vi "Get All Methods.vi"(8 "error in (no error)":errorcluster) -> (0 "error out":errorcluster, 3 "Methods[]":T1(array[cluster]))   [LabVIEW 2023]
panel:
  out "Method Ct":i32
  out "class ct":i32
  out "Data name":string
  out "Class Name (unlocalized)":string
  out "exe time (ms)":u32
  # "After some initial cleanup run time:\n\n70s\n\nAfter a little optimization:\n\n11s"
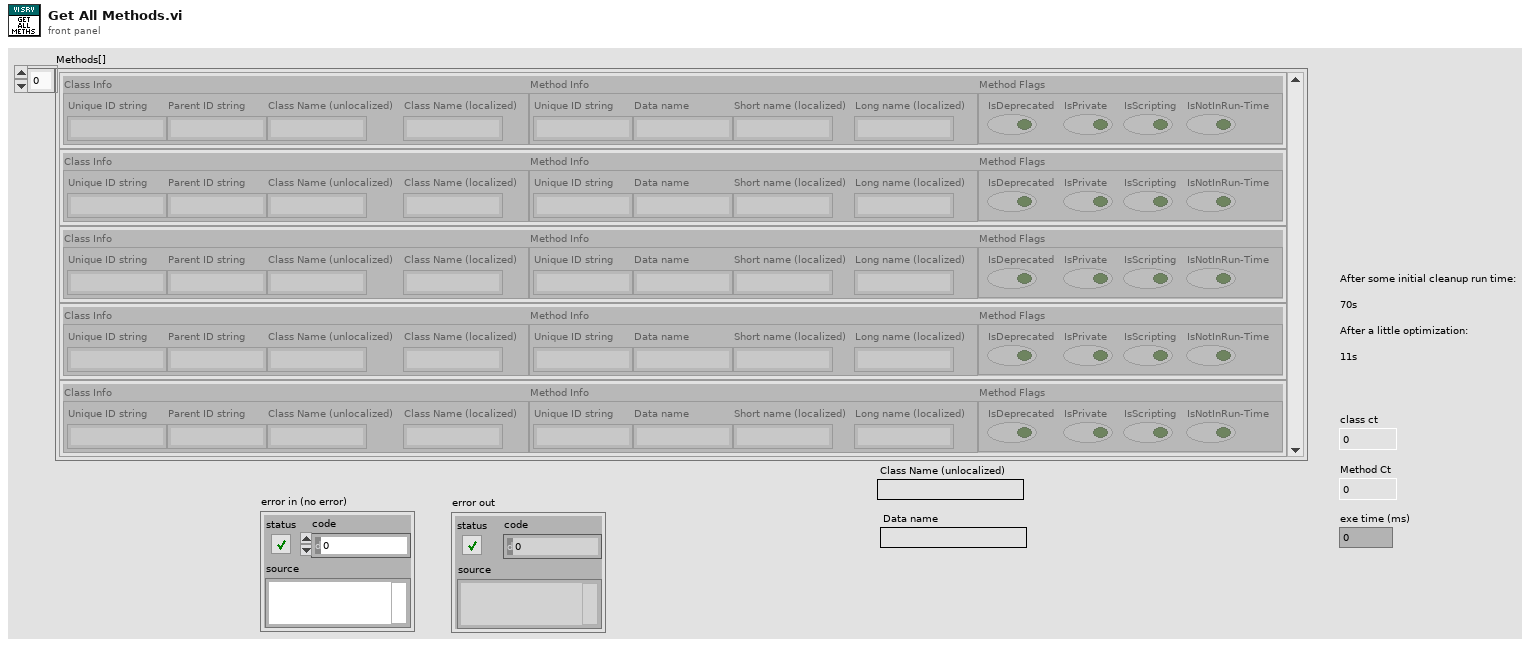
[diagram p1: front panel]
types:
  T1 = cluster{"Class Info":cluster{"Unique ID string":string, "Parent ID string":string, "Class Name (unlocalized)":string, "Class Name (localized)":string}, "Method Info":cluster{"Unique ID string":string, "Data name":string, "Short name (localized)":string, "Long name (localized)":string}, "Method Flags":cluster{"IsDeprecated":bool, "IsPrivate":bool, "IsScripting":bool, "IsNotInRun-Time":bool}}[]
  T2 = cluster{"Unique ID string":string, "Parent ID string":string, "Class Name (unlocalized)":string, "Class Name (localized)":string}[]
  T3 = cluster{"Done":refnum<user-event>, "Msg 1":refnum<user-event>, "Msg 2":refnum<user-event>, "Prog Max":refnum<user-event>, "Prog Ct":refnum<user-event>}
  T4 = cluster{"Property/Method Info":cluster{"Unique ID string":string, "Parent ID string":string, "Class Name (unlocalized)":string, "Class Name (localized)":string}, "Property Info":cluster{"Unique ID string":string, "Data name":string, "Short name (localized)":string, "Long name (localized)":string}, "Method Flags":cluster{"IsDeprecated":bool, "IsPrivate":bool, "IsScripting":bool, "IsNotInRun-Time":bool}}[]
  T5 = cluster{"Unique ID string":string, "Data name":string, "Short name (localized)":string, "Long name (localized)":string}[]
  T6 = cluster{"IsDeprecated":bool, "IsPrivate":bool, "IsScripting":bool, "IsNotInRun-Time":bool}
  T7 = cluster{"Property/Method Info":cluster{"Unique ID string":string, "Parent ID string":string, "Class Name (unlocalized)":string, "Class Name (localized)":string}, "Property Info":cluster{"Unique ID string":string, "Data name":string, "Short name (localized)":string, "Long name (localized)":string}, "Method Flags":cluster{"IsDeprecated":bool, "IsPrivate":bool, "IsScripting":bool, "IsNotInRun-Time":bool}}
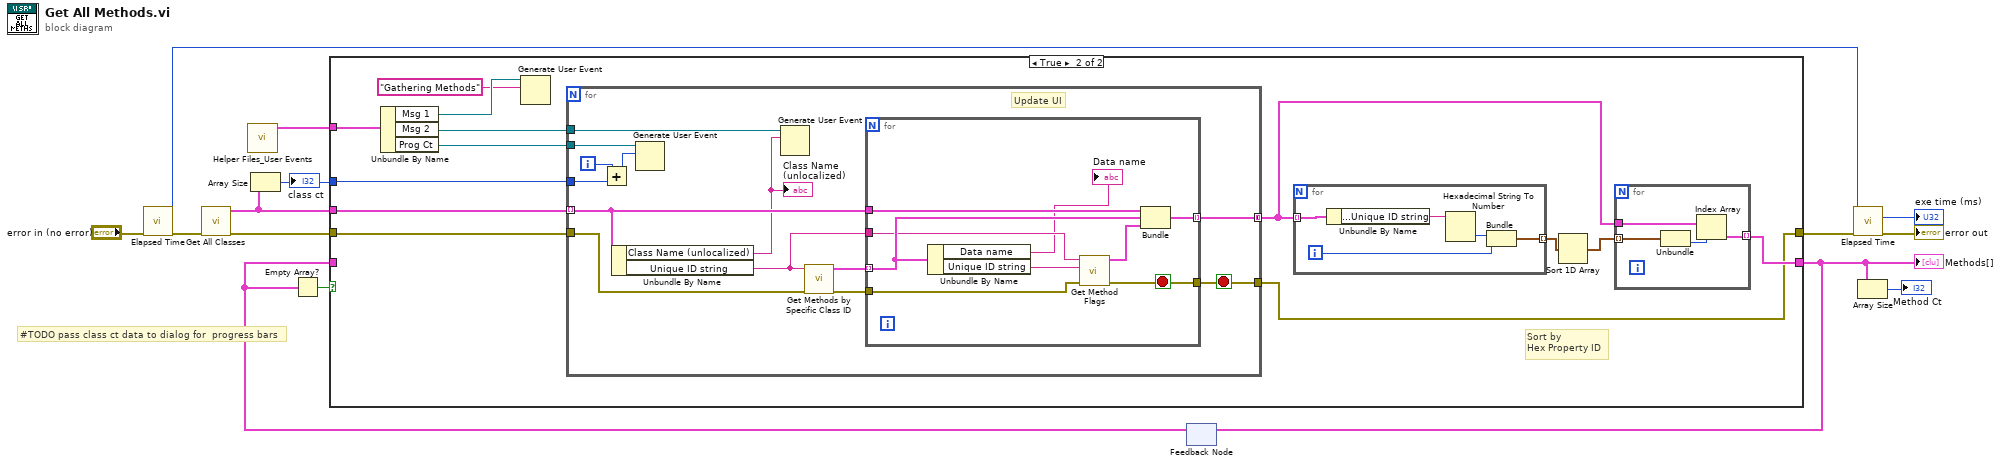
[diagram p0: block diagram]
diagram:
  # "#TODO pass class ct data to dialog for  progress bars"
  n1 = call "Elapsed Time.vi"("error in"="error in (no error)") -> ("error out"=w13:errorcluster, "millisecond timer value"=w8:u32)  [unwired: 6 in, 3 out]
  n2 = call "Get All Classes.vi"("error in (no error)"=w13) -> ("error out"=w6:errorcluster, "VI Server Classes[]"=w5:T2)  [unwired: 9 in]
  n3 = call "Helper Files_User Events.vi"() -> ("Init Dialog UEs"=w2:T3)  [unwired: 11 in]
  n4 = Array Size(array=w5) -> (size(s)=w1:i32)
  "class ct" <- w1
  n5 = feedback #1() -> (w10:T4)  [unwired: 1 in]
  n6 = Empty Array?(array=w10) -> (empty?=w9:bool)
  n7 = case shown="True" w9 {
    tunnel: w5 -> [_ w29]
    tunnel: [w16 w25] -> w4
    tunnel: w10 -> [w16 _]
    tunnel: w6 -> [w15 w24]
    tunnel: [w15 w23] -> w12
    tunnel: w2 -> [_ w22]
    tunnel: w1 -> [_ w17]
    frame False {
    }
    frame True {
      # "Sort by\nHex Property ID"
      n8 = Unbundle By Name(w22) -> ("Msg 1"=w19:refnum<user-event>, "Msg 2"=w21:refnum<user-event>, "Prog Ct"=w20:refnum<user-event>)
      n9 = Generate User Event(user event=w19, event data cluster="Gathering Methods" ("event data")) -> ()  [unwired: 2 in, 2 out]
      n10 = for {
        tunnel: w29 -> [w42] mode=indexing
        tunnel: [w41] -> w26 mode=concatenating
        tunnel: w24 -> [w38]
        tunnel: [w40] -> w23
        tunnel: w21 -> [w35]
        tunnel: w20 -> [w34]
        tunnel: w17 -> [w32]
        i -> [w31]
        stop <- w40 stop-if-true
        # "Update UI"
        n11 = Add(x=w31, y=w32) -> (x+y=w30:i32)
        n12 = Unbundle By Name(w42) -> ("Class Name (unlocalized)"=w33:string, "Unique ID string"=w39:string)
        "Class Name (unlocalized)" <- w33
        n13 = Generate User Event(user event=w34, event data cluster=w30) -> ()  [unwired: 2 in, 2 out]
        n14 = Generate User Event(user event=w35, event data cluster=w33) -> ()  [unwired: 2 in, 2 out]
        n15 = call "Get Methods by Specific Class ID.vi"("error in (no error)"=w38, "Class ID"=w39) -> ("error out"=w37:errorcluster, "Methods[]"=w36:T5)  [unwired: 8 in]
        n16 = for {
          tunnel: w36 -> [w50] mode=indexing
          tunnel: w39 -> [w44]
          tunnel: w42 -> [w51]
          tunnel: [w49] -> w41 mode=indexing
          tunnel: w37 -> [w48]
          tunnel: [w46] -> w40
          stop <- w46 stop-if-true
          n17 = Unbundle By Name(w50) -> ("Data name"=→"Data name":string, "Unique ID string"=w45:string)
          n18 = call "Get Method Flags.vi"("error in (no error)"=w48, "Method ID"=w45, "Class ID"=w44) -> ("error out"=w46:errorcluster, "Method Flags"=w47:T6)  [unwired: 7 in]
          n19 = Bundle("Property/Method Info"=w51, "Property Info"=w50, "Method Flags"=w47) -> (w49:T7)  [unwired: 1 in]
        }
      }
      n20 = for {
        tunnel: [w54] -> w28 mode=indexing
        tunnel: w26 -> [w53] mode=indexing
        i -> [w55]
        n21 = Unbundle By Name(w53) -> ("Property/Method Info.Unique ID string"=w52:string)
        n22 = Hexadecimal String To Number(string=w52) -> (number=w56:u32)  [unwired: 2 in, 1 out]
        n23 = Bundle(w56, w55) -> (w54:cluster{u32, i32})  [unwired: 1 in]
      }
      n24 = Sort 1D Array(array=w28) -> (sorted array=w27:cluster{u32, i32}[])
      n25 = for {
        tunnel: w27 -> [w60] mode=indexing
        tunnel: [w58] -> w25 mode=indexing
        tunnel: w26 -> [w57]
        n26 = Unbundle(w60) -> (w59:i32)  [unwired: 1 out]
        n27 = Index Array(array=w57, index=w59) -> (element=w58:T7)
      }
    }
  }
  "Methods[]" <- w4
  n28 = feedback-in #1(w4) -> ()
  n29 = call "Elapsed Time.vi"("error in"=w12, "past time"=w8) -> ("error out"=→"error out":errorcluster, "elapsed time (ms)"=→"exe time (ms)":u32)  [unwired: 5 in, 3 out]
  n30 = Array Size(array=w4) -> (size(s)=→"Method Ct":i32)
